vi "AlliGator Compute Phasor Plot Phasor Ratio.vi"(4 "State Indicators Refnum":refnum<vi>, 5 "Time Stamp Array":dbl[](array[numeric]), 7 "Phasor Graph":refnum<vi>, 8 "Error In":errorcluster, 9 "Plot Idx":i32, 10 "Phasor Ratio Graph":refnum<vi>, 11 "Lifetime Graph":refnum<vi>) -> (0 "Error Out":errorcluster, 1 "Message":string)   [LabVIEW 2021, in "AlliGator Phasor Ratio.lvlib"]
doc: "Computes phasor ratio and derived quantities and outputs the corresponding plots."
uses:
  AlliGator Phasor Ratio.lvlib
  GUI/AlliGator State Indicator.ctl
  Settings/AlliGator Settings List.ctl
  Phasor/Phasor Ratio Type.ctl
  Phasor/Phasor.lvlib
  Settings/AlliGator Settings+.lvlib
  Graphs/XY Graph/XY Graph Add-Ons.lvlib
  Error/Error.lvlib
  Strings/Strings.lvlib
  Sound/Sound.lvlib
  GUI/AlliGator GUI.lvlib
panel:
  # "see the AlliGator License on the block diagram (Ctrl+E or Window:Show Block Diagram)"
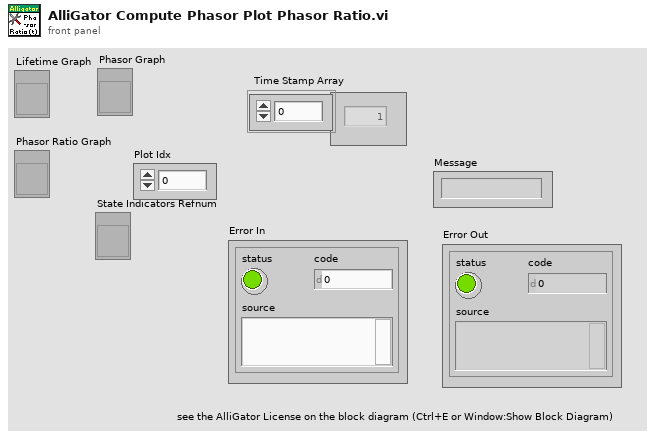
[diagram p1: front panel]
types:
  T1 = typedef "AlliGator State Indicator.ctl" = cluster{"Phasor Calibration Defined":bool, "Phasor Calibration Series Defined":bool, "Phasor Calibration Map Defined":bool, "Phasor Ratio Reference 1 Defined":bool, "Phasor Ratio Reference 2 Defined":bool, "Phasor Ratio Lifetime Reference 1 Defined ":bool, "Phasor Ratio Lifetime Reference 2 Defined":bool, "Phasor Calibration Used":bool, "Phasor Calibration Series Used":bool, "Phasor Calibration Map Used":bool, "Dataset Update Needed":bool, "Phasor Plot Update Needed":bool, "Reference/IRF Defined":bool, "Individual IRFs Defined":bool}
  T2 = typedef "AlliGator Settings+.lvlib/AlliGator Settings List.ctl" = enum16{"GUI:Visible Settings Tab", "GUI:Last Run Version", "Source Image:Use Image Histogram for Contrast", "Source Image:Low Count Pixels Rejection Options", "Source Image:High Count Pixels Rejection Options", "Source Image:Use Image Brightness", "Source Image:Blend Overlay with Image Background", "Source Image:Use Fixed ROI Diameter", "Source Image:ROI Diameter", "Source Image:ROI Center Color", "Source Image:Peak Threshold", "Source Image:Intensity Threshold", "Source Image:Image Binning Options", "Source Image:Image Smoothing Options", "Source Image:Image Histogram Active", "Source Image:Invert Binary Mask", "Source Image:Hot Pixel Removal", "Source Image:Overlay Analyzed ROI Center", "Source Image:Auto-Adjust Contrast", "Source Image:Histogram Lower Percentile", "Source Image:Histogram Upper Percentile", "Source Image:Lock ROI with Maps", "Source Image:Save Source Image", "Source Image:Scale Bar Options", "Source Image:Image Resolution (Pixel Size)", "Source Image:Flatfield Correction", "Source Image:Show Dead Left Columns Correction", "Source Image:Dead Left Columns Correction", "Source Image:Image Pre-Processing Operations Order", "Source Image:Overlay ROI Median", "Source Image:Median Overlay Color", "Data Information:Gate Width", "Data Information:Nanotime Gate Separation", "Data Information:Macrotime Gate Separation", "Data Information:Gate Step", "Data Information:# Gates", "Data Information:Gate Image Exposure", "Data Information:Gate Image Integration", "Data Information:Gates to Skip", "Data Information:Gates to Keep", "Data Information:Define Gates to", "Data Information:Channel Name", "Data Information:Available Channel Names", "Data Information:Channel Arithmetic", "Data Information:Background File Subtraction", "Data Information:Background File", "Data Information:Background Scaling Factor", "Data Information:Background Pile-up Correction", "Data Information:Background Pixel Well Capacity", "Data Information:Laser Period", "Data Information:SYNC Period", "Data Information:Pile-up Correction", "Data Information:Pixel Well Capacity", "Data Information:Dataset Scaling Factor", "Fluorescence Decay_Decay Pre-Processing:Reverse Gates", "Fluorescence Decay_Decay Pre-Processing:Verbose Decay Pre-Processing", "Fluorescence Decay_Decay Pre-Processing:Use Decay Pre-Processing", "Fluorescence Decay_Decay Pre-Processing:Background Subtraction", "Fluorescence Decay_Decay Pre-Processing:Background Definition Range", "Fluorescence Decay_Decay Pre-Processing:Baseline Subtraction Method", "Fluorescence Decay_Decay Pre-Processing:Decay Pre-Processing Operations Order", "Fluorescence Decay_Decay Pre-Processing:Smoothing Parameter", "Fluorescence Decay_Decay Pre-Processing:Shift Decay", "Fluorescence Decay_Decay Pre-Processing:Decay Shift Parameters", "Fluorescence Decay_Decay Pre-Processing:Fold Decay", "Fluorescence Decay_Decay Pre-Processing:# Folds", "Fluorescence Decay_Decay Pre-Processing:1-Normalize Decay", "Fluorescence Decay_Decay Pre-Processing:[0-1]-Normalize Decay", "Fluorescence Decay_Decay Pre-Processing:Smoothen Decay", "Fluorescence Decay_Decay Pre-Processing:Extrapolate Decay", "Fluorescence Decay_Decay Pre-Processing:Use Periodicity", "Fluorescence Decay_Decay Pre-Processing:Use Cursors", "Fluorescence Decay_Decay Pre-Processing:Tail Fraction", "Fluorescence Decay_Decay Pre-Processing:Head Fraction", "Fluorescence Decay_Decay Pre-Processing:Additional Points", "Fluorescence Decay_Decay Pre-Processing:Straighten Decay", "Fluorescence Decay_Decay Pre-Processing:Constant Background", "Fluorescence Decay_Decay Pre-Processing:Pixel-Normalize Decay", "Fluorescence Decay_Advanced Analysis:Extract IRF instead of Decay", "Fluorescence Decay_Advanced Analysis:IRF Extraction Options", "Fluorescence Decay_Advanced Analysis:IRF Optimization Options", "Fluorescence Decay_Advanced Analysis:Square Pulse Options", "Fluorescence Decay_Advanced Analysis:IRF Order", "Fluorescence Decay_Advanced Analysis:IRF Time Constants", "Fluorescence Decay_Advanced Analysis:Wavelet Analysis Options", "Fluorescence Decay_Advanced Analysis:Average Lifetime Options", "Fluorescence Decay_Fit Options:Fit Options", "Fluorescence Decay_Fit Options:Use Legacy Fitting Approach", "Fluorescence Decay_Fit Options:Use Data Information Laser Period", "Fluorescence Decay_Fit Parameters:Displayed Fit Parameters", "Fluorescence Decay_Fit Parameters:Fit Parameter Constraints", "Fluorescence Decay_Fit Parameters:Export Tabulated Results", "Fluorescence Decay_Fit Parameters:MLE Baseline Offset Type", "Fluorescence Decay_Fit Parameters:MLE Baseline Offset", "Fluorescence Decay_Fit Parameters:Guess Parameter Names", "Fluorescence Decay_Fit Parameters:Guess Parameter Values", "Fluorescence Decay_Fit Parameters:Guess Parameters Options", "Fluorescence Decay_Fit Parameters:Optimal Offset Selection Criterion", "Fluorescence Decay_Styles:Show Last Decay Only", "Fluorescence Decay_Styles:Decay Graph Color Array", "Fluorescence Decay:Decay Graph Active", "Fluorescence Decay Statistics:Min Peak Value", "Fluorescence Decay Statistics:Reject Low Decay Peak Pixels", "Fluorescence Decay Statistics:Reject High Decay Peak Pixels", "Fluorescence Decay Statistics:Max Peak Value", "Time Traces:Use File Timestamp", "Time Traces:Time Step", "Time Traces:Use Intensity Correction File", "Time Traces:Intensity Correction File", "Phasor Plot:Phasor Plot Smoothing Options", "Phasor Plot:Phasor Plot Size", "Phasor Plot:Phasor Plot Graphics Options", "Phasor Plot:Cumulative Phasor Plot", "Phasor Plot:Use Phasor Brightness", "Phasor Plot:Blend Overlay with Phasor Background", "Phasor Plot:Save Phasor Plot", "Phasor Plot:Show References", "Phasor Plot:Phasor Ratio Decay Range", "Phasor Plot:Exponential Fading", "Phasor Plot:Phasor Ratio Reference Colors", "Phasor Plot:Reference Radius", "Phasor Plot:Show Color Map Vertices", "Phasor Plot:Phasor Plot Active", "Phasor Plot:Phasor Ratio Color Map Type", "Phasor Plot:Phasor Ratio Color Map", "Phasor Plot:Phasor Ratio Display Range", "Phasor Plot:Selected Image ROI(s)", "Phasor Plot:All Image ROIs", "Phasor Plot:Selected Phasor Plot ROI(s)", "Phasor Plot:All Phasor Plot ROIs", "Phasor Plot:Phasor Ratio Color-Coded Quantity", "Phasor Plot:Store Phasor Harmonics", "Phasor Plot:Draw Reference Segment", "Phasor Plot:User-Defined Quantity", "Phasor Plot:Color Scale High Color", "Phasor Plot:Color Scale Low Color", "Phasor Plot:Intensity-weighted Phasor Plot", "Phasor Graph:Phasor Frequency", "Phasor Graph:Phasor Ratio Type", "Phasor Graph:Pixel-level Phasor Computation", "Phasor Graph:Save Phasor Graph", "Phasor Graph:Phasor Graph Active", "Phasor Graph:Phasor SDV Options", "Phasor Graph:Intensity-weighted Phasor Graph", "Phasor Graph:Define Shortest Lifetime as", "Phasor Calibration:Use Backup Calibration if needed", "Phasor Calibration:Backup Calibration Type", "Phasor Calibration:Calibration Type", "Phasor Calibration:Calibration Lifetime", "Phasor Calibration:Calibration Map Algorithm", "Single-Exponential Phasor Locus (SEPL):Gate Parameters", "Single-Exponential Phasor Locus (SEPL):User-defined Gate", "Single-Exponential Phasor Locus (SEPL):User-defined IRF", "Single-Exponential Phasor Locus (SEPL):Phasor Parameters", "Single-Exponential Phasor Locus (SEPL):Decay & IRF Parameters", "Single-Exponential Phasor Locus (SEPL):Display Parameters", "Lifetime Analysis:Decay Analysis Parameters", "Lifetime Analysis:Lifetime Map Active", "Plugins:Python Settings", "Miscellaneous:Verbose Mode", "Miscellaneous:Beep after Script", "Miscellaneous:Saved Image File Format", "Miscellaneous:Exported Gate Image Settings", "Miscellaneous:Include Loading in Timing", "Miscellaneous:Verbose Settings Mode", "Miscellaneous:Histogram Options", "Miscellaneous:Beep on Error", "Miscellaneous:# Logical Processors Used", "Miscellaneous:ROI Description Max Characters", "Miscellaneous:Verbose Error Mode", "Miscellaneous:Transparent Mask Color"}
  T3 = typedef "Phasor.lvlib/Phasor Ratio Type.ctl" = enum32{"Intensity-weighted", "Amplitude-weighted"}
  T4 = typedef "Phasor.lvlib/Phasor (g, s).ctl" = cluster{"g":dbl, "s":dbl}
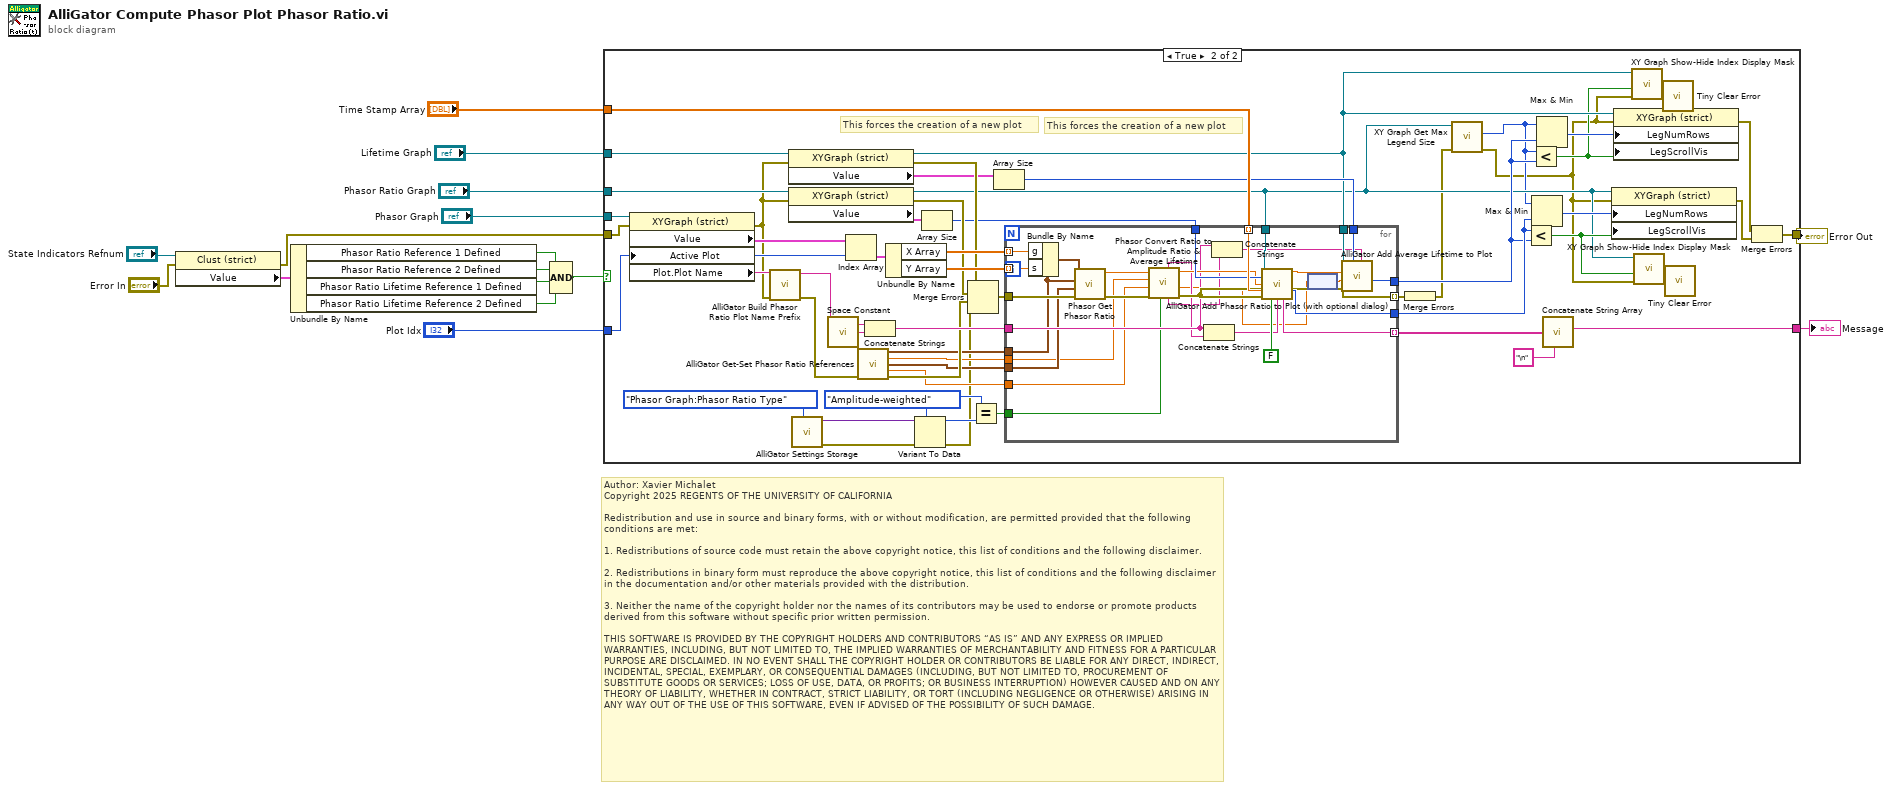
[diagram p0: block diagram]
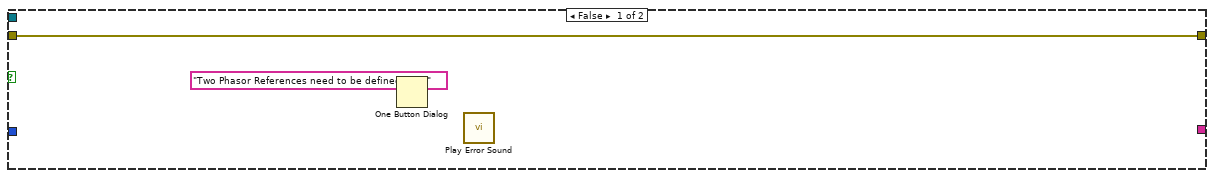
[diagram p2: hidden frame]
diagram:
  # "Author: Xavier Michalet\nCopyright 2025 REGENTS OF THE UNIVERSITY OF CALIFORNIA\n\nRedistribution and use in source and binary forms, with or without modification, are permitted provided that the following conditions are met:\n\n1. Redistributions of source code must retain the above copyright notice, this list of conditions and the following disclaimer.\n\n2. Redistributions in binary form must reproduce the above copyright notice, this list of conditions and the following disclaimer in the documentation and/or other materials provided with the distribution.\n\n3. Neither the name of the copyright holder nor the names of its contributors may be used to endorse or promote products derived from this software without specific prior written permission.\n\nTHIS SOFTWARE IS PROVIDED BY THE COPYRIGHT HOLDERS AND CONTRIBUTORS “AS IS” AND ANY EXPRESS OR IMPLIED WARRANTIES, INCLUDING, BUT NOT LIMITED TO, THE IMPLIED WARRANTIES OF MERCHANTABILITY AND FITNESS FOR A PARTICULAR PURPOSE ARE DISCLAIMED. IN NO EVENT SHALL THE COPYRIGHT HOLDER OR CONTRIBUTORS BE LIABLE FOR ANY DIRECT, INDIRECT, INCIDENTAL, SPECIAL, EXEMPLARY, OR CONSEQUENTIAL DAMAGES (INCLUDING, BUT NOT LIMITED TO, PROCUREMENT OF SUBSTITUTE GOODS OR SERVICES; LOSS OF USE, DATA, OR PROFITS; OR BUSINESS INTERRUPTION) HOWEVER CAUSED AND ON ANY THEORY OF LIABILITY, WHETHER IN CONTRACT, STRICT LIABILITY, OR TORT (INCLUDING NEGLIGENCE OR OTHERWISE) ARISING IN ANY WAY OUT OF THE USE OF THIS SOFTWARE, EVEN IF ADVISED OF THE POSSIBILITY OF SUCH DAMAGE."
  n1 = property class="Clust (strict)"(reference="State Indicators Refnum", error in="Error In") -> (error out=w2:errorcluster, "Value"=w4:T1)  [unwired: 1 out]
  n2 = Unbundle By Name(w4) -> ("Phasor Ratio Reference 1 Defined"=w14:bool, "Phasor Ratio Reference 2 Defined"=w13:bool, "Phasor Ratio Lifetime Reference 1 Defined"=w12:bool, "Phasor Ratio Lifetime Reference 2 Defined"=w11:bool)
  n3 = Compound Arithmetic op=AND(w14, w13, w12, w11) -> (w10:bool)
  n4 = case shown="True" w10 {
    tunnel: "Lifetime Graph" -> [_ w73]
    tunnel: "Phasor Ratio Graph" -> [_ w72]
    tunnel: w2 -> [w17 w70]
    tunnel: [w17 w40] -> w9
    tunnel: "Phasor Graph" -> [_ w71]
    tunnel: "Time Stamp Array" -> [_ w63]
    tunnel: "Plot Idx" -> [_ w52]
    tunnel: [_ w24] -> w1
    frame False {
      n5 = One Button Dialog(message="Two Phasor References need to be defined first!") -> ()  [unwired: 1 in, 1 out]
      n6 = call "Play Error Sound.vi"() -> ()  [unwired: 27 in, 1 out]
    }
    frame True {
      w30 = Phasor_Ratio_Type."Amplitude-weighted" ("Phasor Ratio Type")
      # "This forces the creation of a new plot"
      # "This forces the creation of a new plot"
      n7 = property class="XYGraph (strict)"(reference=w71, error in=w70, "Active Plot"=w52) -> (error out=w47:errorcluster, "Value"=w61:cluster{"X Array":dbl[], "Y Array":dbl[]}[], "Plot.Plot Name"=w51:string)  [unwired: 1 out]
      n8 = call "AlliGator Build Phasor Ratio Plot Name Prefix.vi"("Error In"=w47, "Phasor Plot Name in"=w51) -> ("Error Out"=w46:errorcluster, "Phasor Ratio Plot Name Prefix out"=w50:string)  [unwired: 8 in]
      n9 = property class="XYGraph (strict)"(reference=w73, error in=w47) -> (reference out=w33:refnum<vi>, error out=w66:errorcluster, "Value"=w59:cluster{"X Array":dbl[], "Y Array":dbl[]}[])
      n10 = property class="XYGraph (strict)"(reference=w72, error in=w47) -> (reference out=w22:refnum<vi>, error out=w65:errorcluster, "Value"=w62:cluster{"X Array":dbl[], "Y Array":dbl[]}[])
      n11 = call "AlliGator Settings Storage.vi"("AlliGator Settings List"=AlliGator_Settings_List."Phasor Graph:Phasor Ratio Type") -> ("Error Out"=w28:errorcluster, "Variant Data out"=w29:variant)  [unwired: 9 in]
      n12 = call <vilib>:"Space Constant.vi"() -> ("String"=w48:string)
      n13 = Index Array(array=w61, index=w52) -> (element=w69:cluster{"X Array":dbl[], "Y Array":dbl[]})
      n14 = call "AlliGator Get-Set Phasor Ratio References.vi"("error in (no error)"=w46) -> ("Reference Phasor 1"=w44:T4, "Reference Lifetime 1"=w42:dbl[unit], "Reference Phasor 2"=w43:T4, "Reference Lifetime 2"=w41:dbl[unit], "error out"=w45:errorcluster)  [unwired: 7 in, 3 out]
      n15 = Concatenate Strings(w50, w48) -> (w49:string)
      n16 = Unbundle By Name(w69) -> ("X Array"=w68:dbl[], "Y Array"=w67:dbl[])
      n17 = Variant To Data(error in=w28, type=w30, Variant=w29) -> (data=w31:T3, error out=w26:errorcluster)
      n18 = Array Size(array=w62) -> (size(s)=w60:i32)
      n19 = Merge Errors(w66, w65, w45, w26) -> (w64:errorcluster)
      n20 = Equal?(x=w30, y=w31) -> (x = y?=w27:bool)
      n21 = Array Size(array=w59) -> (size(s)=w58:i32)
      n22 = for {
        tunnel: w33 -> [w104]
        tunnel: w22 -> [w103]
        tunnel: w68 -> [w100] mode=indexing
        tunnel: w67 -> [w99] mode=indexing
        tunnel: w63 -> [w96] mode=indexing
        tunnel: w60 -> [w95]
        tunnel: w58 -> [w94]
        tunnel: [w93] -> w54
        tunnel: [w92] -> w53
        tunnel: w49 -> [w86]
        tunnel: w64 -> [w101]
        tunnel: [w84] -> w57 mode=indexing
        tunnel: w44 -> [w83]
        tunnel: w43 -> [w82]
        tunnel: w42 -> [w80]
        tunnel: w41 -> [w79]
        tunnel: w27 -> [w77]
        tunnel: [w76] -> w25 mode=indexing
        n23 = Bundle By Name(cluster=w83, "g"=w100, "s"=w99) -> (w98:T4)
        n24 = call "Phasor Get Phasor Ratio.vi"("Error In"=w101, "Reference Phasor 2"=w82, "Reference Phasor 1"=w83, "Phasor"=w98) -> ("Error Out"=w90:errorcluster, "Phasor Ratio (f1)"=w91:dbl)  [unwired: 5 in, 1 out]
        n25 = call "Phasor Convert Ratio to Amplitude Ratio & Average Lifetime.vi"("Compute Amplitude Ratio"=w77, "error in (no error)"=w90, "Reference Lifetime 2"=w79, "Reference Lifetime 1"=w80, "Phasor Ratio (f1)"=w91) -> ("error out"=w89:errorcluster, "Average Lifetime"=w75:dbl[unit], "Phasor/Amplitude Ratio"=w88:dbl, "Average Lifetime Caption"=w78:string, "Phasor Ratio Plot Name Suffix"=w81:string)  [unwired: 2 in]
        n26 = Concatenate Strings(w86, w81) -> (w87:string)
        n27 = Concatenate Strings(w86, w78) -> (w85:string)
        n28 = call "AlliGator Add Phasor Ratio to Plot (with optional dialog).vi"("XYGraph in"=w103, "Plot ID (-1)"=w95, "Phasor Ratio"=w88, "Time Point"=w96, "error in (no error)"=w89, "Interactive?"=FALSE, "New Plot Name"=w87) -> ("Sample Abscissa"=w102:dbl, "# Plots"=w93:i32, "Message"=w76:string)  [unwired: 3 in, 3 out]
        n29 = node(w75) -> (w74:dbl)
        n30 = call "AlliGator Add Average Lifetime to Plot.vi"("New Plot Name"=w85, "Plot ID (-1)"=w94, "error in (no error)"=w89, "Average Lifetime"=w74, "Abscissa"=w102, "Lifetime Graph refnum"=w104) -> ("error out"=w84:errorcluster, "# Plots"=w92:i32)  [unwired: 2 in, 2 out]
      }
      n31 = Merge Errors(w57) -> (w20:errorcluster)
      n32 = call "XY Graph Get Max Legend Size.vi"("Error In"=w20, "XYGraph Refnum"=w22) -> ("Error Out"=w19:errorcluster, "Max Legend Size"=w21:i32)  [unwired: 6 in, 2 out]
      n33 = Less?(x=w54, y=w53) -> (x < y?=w35:bool)
      n34 = Less?(x=w21, y=w53) -> (x < y?=w32:bool)
      n35 = Max & Min(x=w21, y=w54) -> (min(x,y)=w55:i32)  [unwired: 1 out]
      n36 = Max & Min(x=w21, y=w53) -> (min(x,y)=w56:i32)  [unwired: 1 out]
      n37 = call "Concatenate String Array.vi"("Separator (TAB)"="\n", "String Array"=w25) -> ("Formatted String"=w24:string)  [unwired: 9 in]
      n38 = property class="XYGraph (strict)"(reference=w22, error in=w19, "LegNumRows"=w55, "LegScrollVis"=w35) -> (error out=w38:errorcluster)  [unwired: 1 out]
      n39 = property class="XYGraph (strict)"(reference=w33, error in=w19, "LegNumRows"=w56, "LegScrollVis"=w32) -> (error out=w39:errorcluster)  [unwired: 1 out]
      n40 = call "XY Graph Show-Hide Index Display Mask.vi"("error in (no error)"=w19, "Show(T)/Hide(F)"=w32, "XYGraph Ref"=w33) -> ("error out"=w34:errorcluster)  [unwired: 7 in, 1 out]
      n41 = call "XY Graph Show-Hide Index Display Mask.vi"("error in (no error)"=w19, "Show(T)/Hide(F)"=w35, "XYGraph Ref"=w22) -> ("error out"=w36:errorcluster)  [unwired: 7 in, 1 out]
      n42 = call "Tiny Clear Error.vi"("Error In"=w34) -> ()  [unwired: 8 in, 1 out]
      n43 = call "Tiny Clear Error.vi"("Error In"=w36) -> ()  [unwired: 8 in, 1 out]
      n44 = Merge Errors(w39, w38) -> (w40:errorcluster)
    }
  }
  "Error Out" <- w9
  "Message" <- w1
